vi "AddChannel.vi"(8 "error in (no error)":errorcluster, 10 "Channel":refnum<class "Channel.lvclass">, 11 "object in":refnum<class "ChannelManagerUI.lvclass">) -> (0 "error out":errorcluster, 3 "object out":refnum<class "ChannelManagerUI.lvclass">)   [LabVIEW 2021, in "Channel.lvlib" / "ChannelManagerUI.lvlib" / "ChannelManagerUI.lvclass"]
doc: "Adds the channel"
uses:
  ChannelManagerUI.lvclass
  Channel_class/Channel.lvclass
  ChannelsManager/ChannelsManager/ChannelsManager.lvclass
  ChannelManagerUI.lvclass/ChannelManagerUI.ctl
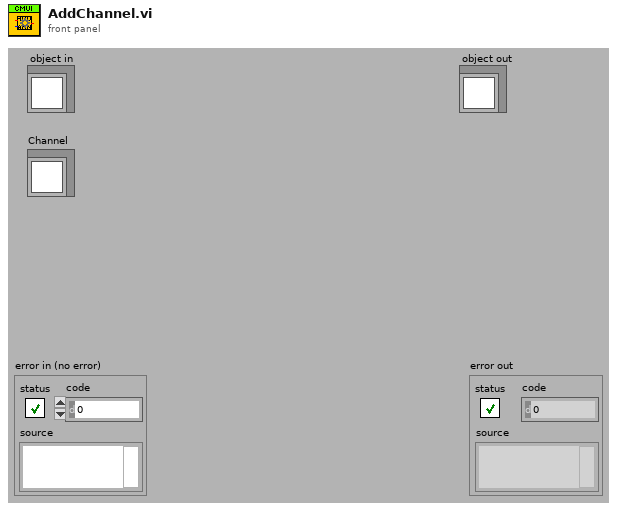
[diagram p1: front panel]
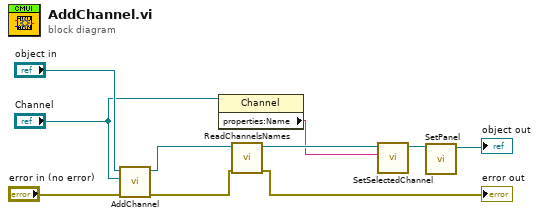
[diagram p0: block diagram]
diagram:
  n1 = call-parent "AddChannel.vi"("error in (no error)"="error in (no error)", "Channel"="Channel", "object in"="object in") -> ("error out"=w7:errorcluster, "object out"=w10:refnum<class "ChannelManagerUI.lvclass">)  [unwired: 7 in]
  n2 = property class="Channel"(reference="Channel") -> ("properties:Name"=w1:string)  [unwired: 1 in, 2 out]
  n3 = call-dynamic "ReadChannelsNames.vi"("error in (no error)"=w7, "ChannelManagerUI in"=w10) -> ("error out"=→"error out":errorcluster, "ChannelManagerUI out"=w3:refnum<class "ChannelManagerUI.lvclass">)  [unwired: 7 in, 1 out]
  n4 = call-dynamic "SetSelectedChannel.vi"("Channel Name"=w1, "object in"=w3) -> ("object out"=w4:refnum<class "ChannelManagerUI.lvclass">)  [unwired: 8 in, 1 out]
  n5 = call-dynamic "SetPanel.vi"("ChannelManagerUI in"=w4) -> ("ChannelManagerUI out"=→"object out":refnum<class "ChannelManagerUI.lvclass">)  [unwired: 9 in, 1 out]
